vi "ISO8601 DateString to Timestamp.vi"(8 "deprecated":bool=TRUE, 9 "Strict ISO? (T)":bool=TRUE, 11 "ISO8601 String":string) -> (1 "valid?":bool, 2 "ISO Format":T1, 3 "Timestamp":timestamp)   [LabVIEW 2013]
doc: "Use \"ISO8601 String to Timestamp.vi\" as a drop-in replacement.\n\nThe VI is kept for backward compatibility, but is deprecated due to confusing name."
uses:
  ISO8601 Date Formats.ctl
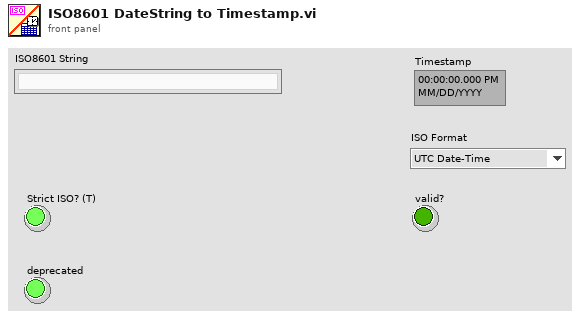
[diagram p1: front panel]
types:
  T1 = typedef "ISO8601 Date Formats.ctl" = enum16{"UTC Date-Time", "ISO Time", "Date", "Calendar Month", "Week", "Week-Day", "Month-Day", "Ordinal Date"}
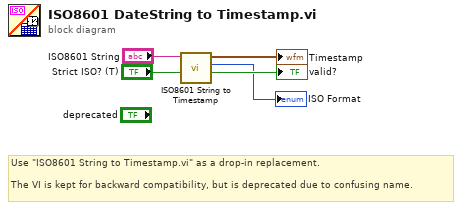
[diagram p0: block diagram]
diagram:
  # "Use \"ISO8601 String to Timestamp.vi\" as a drop-in replacement.\n\nThe VI is kept for backward compatibility, but is deprecated due to confusing name."
  n1 = call "ISO8601 String to Timestamp.vi"("Strict ISO? (T)"="Strict ISO? (T)", "ISO8601 String"="ISO8601 String") -> ("valid?"=→"valid?":bool, "ISO Format"=→"ISO Format":T1, "Timestamp"=→"Timestamp":timestamp)  [unwired: 7 in]
